vi "Sort Wire Terminals into Joint Order.vi"(8 "Error IO":errorcluster, 9 "Terminal Joint Indices":i32[](array[numeric]), 11 "Wire Refnum":refnum<vi>) -> (0 "Error Out":errorcluster, 1 "Sorted Pointers Out":i32[](array[numeric]), 2 "Sorted Terminals Out":refnum<vi>[](array[refnum]), 3 "Wire Refnum Out":refnum<vi>)   [LabVIEW 2012, in "Scripting Tools.lvlib"]
doc: "Resorts the terminals[] property of a wre into the same order that the terminating joints of the wire run. The source terminal will still be the first terminal and the sinks follow. Terminals are matched to joints in the wire on the basis of being closest because there doesn't appear to be a better algorithm."
uses:
  Scripting Tools.lvlib
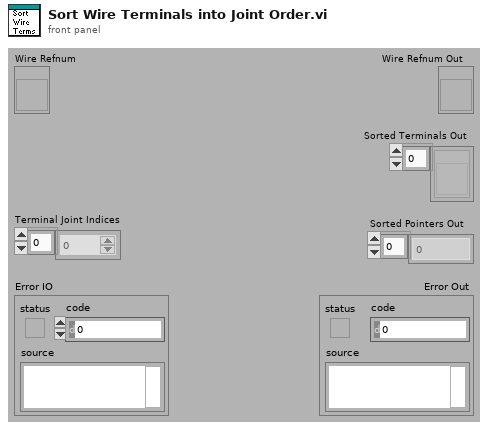
[diagram p1: front panel]
types:
  T1 = cluster{"Position":cluster{"h":i16, "v":i16}, "Flags":i32, "Type":enum32{"LooseEnd", "Endpoint", "Bend", "Junction"}, "Up Joint Index":i16, "Down Joint Index":i16, "Left Joint Index":i16, "Right Joint Index":i16}[]
  T2 = typedef "LVPositionTypeDef.ctl" = cluster{"Left":i32, "Top":i32}
  T3 = cluster{"Position":cluster{"h":i16, "v":i16}, "Flags":i32, "Type":enum32{"LooseEnd", "Endpoint", "Bend", "Junction"}, "Up Joint Index":i16, "Down Joint Index":i16, "Left Joint Index":i16, "Right Joint Index":i16}
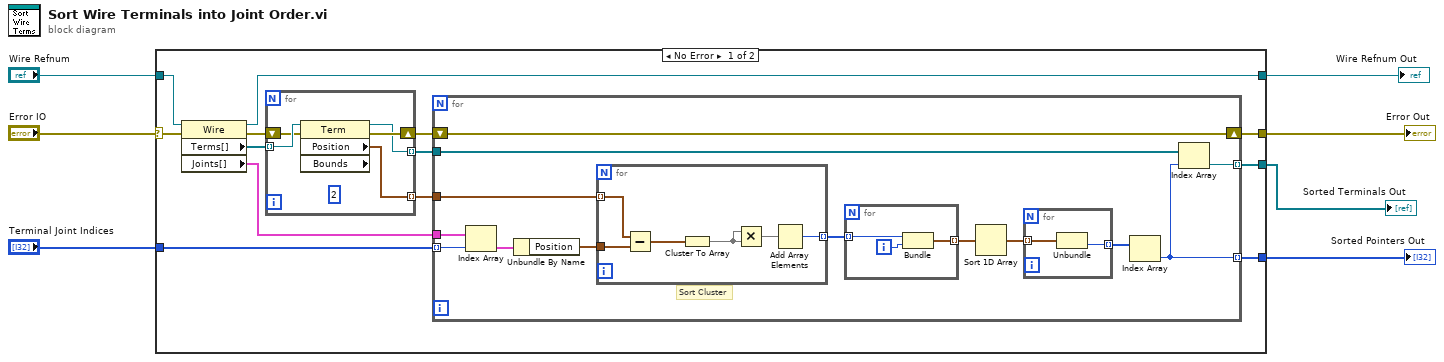
[diagram p0: block diagram]
diagram:
  n1 = case shown="No Error" "Error IO" {
    selector: "Error IO" -> [w8 w51]
    tunnel: [w18 w51] -> w7
    tunnel: [w17 _] -> w6
    tunnel: "Terminal Joint Indices" -> [w15 _]
    tunnel: "Wire Refnum" -> [w12 w50]
    tunnel: [w11 w50] -> w3
    tunnel: [w9 _] -> w2
    frame No Error {
      n2 = property class="Wire"(reference=w12, error in=w8) -> (reference out=w11:refnum<vi>, error out=w19:errorcluster, "Terms[]"=w20:refnum<vi>[], "Joints[]"=w13:T1)
      n3 = for {
        tunnel: w20 -> [w49] mode=indexing
        tunnel: [w48] -> w14 mode=indexing
        shift-right: [w47] -> w16
        shift-left: w19 -> [w46]
        tunnel: [w45] -> w10 mode=indexing
        (unwired) 2
        n4 = property class="Term" props=["Position", "Bounds"](reference=w49, error in=w46) -> (reference out=w45:refnum<vi>, error out=w47:errorcluster, "Position"=w48:T2)  [unwired: 1 out]
      }
      n5 = for {
        tunnel: w15 -> [w33] mode=indexing
        tunnel: w13 -> [w32]
        tunnel: w14 -> [w29]
        tunnel: [w27] -> w17 mode=indexing
        shift-right: [w28] -> w18
        shift-left: w16 -> [w28]
        tunnel: w10 -> [w26]
        tunnel: [w25] -> w9 mode=indexing
        # "Sort Cluster"
        n6 = Index Array(array=w32, index=w33) -> (element=w31:T3)
        n7 = Unbundle By Name(w31) -> ("Position"=w30:cluster{"h":i16, "v":i16})
        n8 = for {
          tunnel: w30 -> [w44]
          tunnel: w29 -> [w43] mode=indexing
          tunnel: [w39] -> w22 mode=indexing
          n9 = Subtract(x=w43, y=w44) -> (x-y=w42:T2)
          n10 = Cluster To Array(cluster=w42) -> (array=w41:i32[])
          n11 = Multiply(x=w41, y=w41) -> (x*y=w40:i32[])
          n12 = Add Array Elements(numeric array=w40) -> (sum=w39:i32)
        }
        n13 = for {
          tunnel: w22 -> [w36] mode=indexing
          tunnel: [w34] -> w23 mode=indexing
          i -> [w35]
          n14 = Bundle("Left"=w36, w35) -> (w34:cluster{"Left":i32, i32})  [unwired: 1 out]
        }
        n15 = Sort 1D Array(array=w23) -> (sorted array=w24:cluster{"Left":i32, i32}[])
        n16 = for {
          tunnel: w24 -> [w38] mode=indexing
          tunnel: [w37] -> w21 mode=indexing
          n17 = Unbundle(w38) -> (w37:i32)  [unwired: 1 out]
        }
        n18 = Index Array(array=w21) -> (element=w27:i32)  [unwired: 1 in]
        n19 = Index Array(array=w26, index=w27) -> (element=w25:refnum<vi>)
      }
    }
    frame Error {
    }
  }
  "Error Out" <- w7
  "Sorted Pointers Out" <- w6
  "Sorted Terminals Out" <- w2
  "Wire Refnum Out" <- w3
